vi "Speed_Feedback.vi"(8 "error in (no error)":errorcluster, 11 "Motor in":refnum<class "Motor.lvclass">) -> (0 "error out":errorcluster, 2 "Actual Speed":dbl, 3 "Motor out":refnum<class "Motor.lvclass">)   [LabVIEW 2021, in "Motor.lvclass"]
uses:
  Motor.lvclass
  Motor.lvclass/Motor.ctl
  AnalogInput/AnalogInput.lvclass
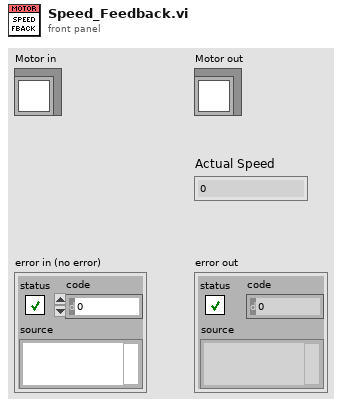
[diagram p1: front panel]
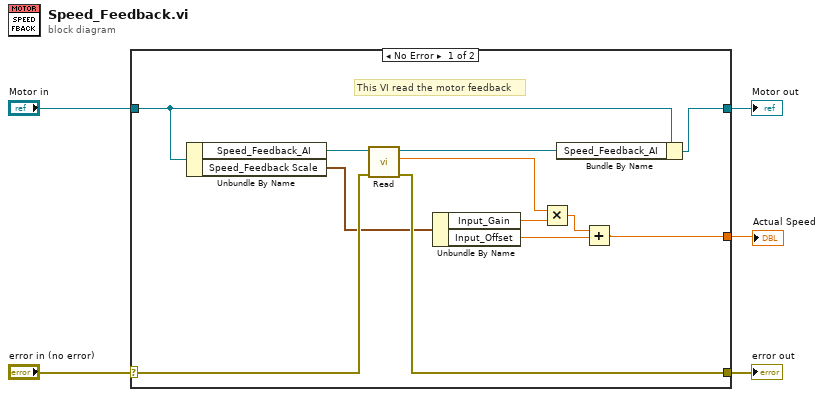
[diagram p0: block diagram]
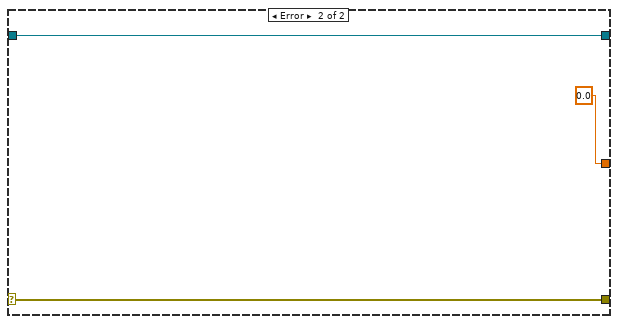
[diagram p2: hidden frame]
diagram:
  n1 = case shown="No Error" "error in (no error)" {
    selector: "error in (no error)" -> [w17 w20]
    tunnel: [w15 w20] -> w4
    tunnel: [w12 w19] -> w2
    tunnel: "Motor in" -> [w14 w19]
    tunnel: [w6 0.0 ("Data Out")] -> w1
    frame No Error {
      # "This VI read the motor feedback"
      n2 = Unbundle By Name(w14) -> ("Speed_Feedback_AI"=w16:refnum<class "AnalogInput.lvclass">, "Speed_Feedback Scale"=w11:cluster{"Input_Gain":dbl, "Input_Offset":dbl})
      n3 = call-dynamic "Read.vi"("error in (no error)"=w17, "AnalogInput in"=w16) -> ("error out"=w15:errorcluster, "Data Out"=w9:dbl, "AnalogInput out"=w13:refnum<class "AnalogInput.lvclass">)  [unwired: 7 in]
      n4 = Unbundle By Name(w11) -> ("Input_Gain"=w10:dbl, "Input_Offset"=w7:dbl)
      n5 = Multiply(x=w9, y=w10) -> (x*y=w8:dbl)
      n6 = Bundle By Name(cluster=w14, "Speed_Feedback_AI"=w13) -> (w12:refnum<class "Motor.lvclass">)
      n7 = Add(x=w8, y=w7) -> (x+y=w6:dbl)
    }
    frame Error {
    }
  }
  "error out" <- w4
  "Motor out" <- w2
  "Actual Speed" <- w1
